vi "ZM-HW-do.vi"(8 "error in (no error)":errorcluster, 11 "ZM-HW-hardware in":refnum<class "ZM-HW-SIM-simulated_hardware.lvclass">) -> (0 "error out":errorcluster, 2 "package":refnum<class "ZM-PC-package.lvclass">, 3 "ZM-HW-hardware out":refnum<class "ZM-HW-SIM-simulated_hardware.lvclass">)   [LabVIEW 2020, in "ZM-HW-SIM-simulated_hardware.lvlib" / "ZM-HW-SIM-simulated_hardware.lvclass"]
doc: "The simulated hardware's ZM-HW-do: makes random test data (ZM-HW-SIM-randomData), wraps it in a test package addressed to Communication and returns it as a ZM-PC-package. No Call Parent."
uses:
  ZM-HW-SIM-simulated_hardware.lvclass
  common/ZM-PC-packages/ZM-PC-package/ZM-PC-package.lvclass
  common/ZM-PC-packages/ZM-PC-TP-test_package/ZM-PC-TP-test_package.lvclass
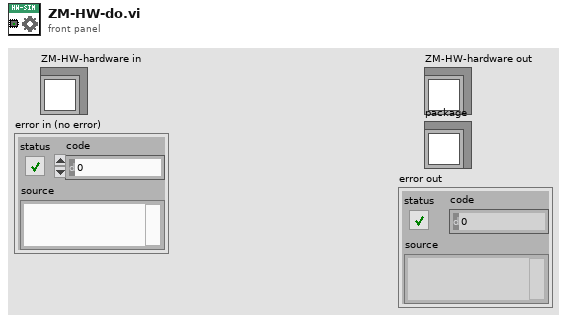
[diagram p1: front panel]
types:
  T1 = enum16{"Unknown", "Root", "Hardware", "Communication"}
  T2 = typedef "ZM-PC-packages.lvlib/ZM-PC-TP-test_package.lvclass/ZM-PC-TP-DATA.ctl" = cluster{"temperature_c":dbl, "sample_index":i32, "duty_percent":u8, "sensor_ok":bool, "status":string}
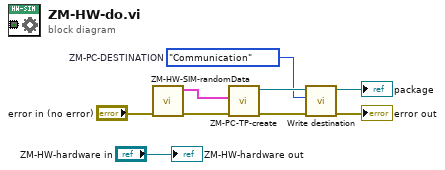
[diagram p0: block diagram]
diagram:
  w4 = T1."Communication"  # ZM-PC-DESTINATION
  n1 = call "ZM-HW-SIM-randomData.vi"("error in (no error)"="error in (no error)") -> ("error out"=w7:errorcluster, "data"=w8:T2)  [unwired: 9 in]
  n2 = call "ZM-PC-TP-create.vi"("error in (no error)"=w7, "data"=w8) -> ("error out"=w6:errorcluster, "package"=w5:refnum<class "ZM-PC-TP-test_package.lvclass">)  [unwired: 8 in]
  n3 = call "Write destination.vi"("error in (no error)"=w6, "ZM-PC-DESTINATION"=w4, "ZM-PC-package in"=w5) -> ("error out"=→"error out":errorcluster, "ZM-PC-package out"=→"package":refnum<class "ZM-PC-TP-test_package.lvclass">)  [unwired: 7 in]
  "ZM-HW-hardware out" <- "ZM-HW-hardware in"
